vi "Check Action.vi"(6 "HRS Time":dbl, 7 "Values In":dbl[](array[numeric]), 8 "error in (no error)":errorcluster, 11 "Valve in":refnum<class "BangBangControl.lvclass">) -> (0 "error out":errorcluster, 2 "Actions":T1[](array[typedef]), 3 "Valve out":refnum<class "BangBangControl.lvclass">, 5 "Values":dbl[](array[numeric]))   [LabVIEW 2020, in "VolatusControl.lvlib" / "BangBangControl.lvclass"]
uses:
  BangBangControl.lvclass
  Control Action.ctl
  Volatus/MessageQ/MessageQ.lvclass
  BangBangControl.lvclass/BangBangControl.ctl
  State.ctl
  PV Calc/PV Calc.lvclass
  VolatusControl.lvlib
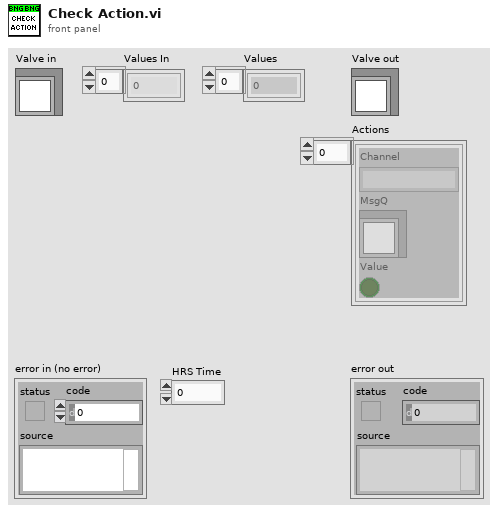
[diagram p1: front panel]
types:
  T1 = typedef "VolatusControl.lvlib/Control Action.ctl" = cluster{"Channel":string, "MsgQ":refnum<class "MessageQ.lvclass">, "Value":bool}
  T2 = typedef "VolatusControl.lvlib/BangBangControl.lvclass/State.ctl" = enum16{"Idle", "RampUp", "RampDown", "Hold", "Disable", "Enable"}
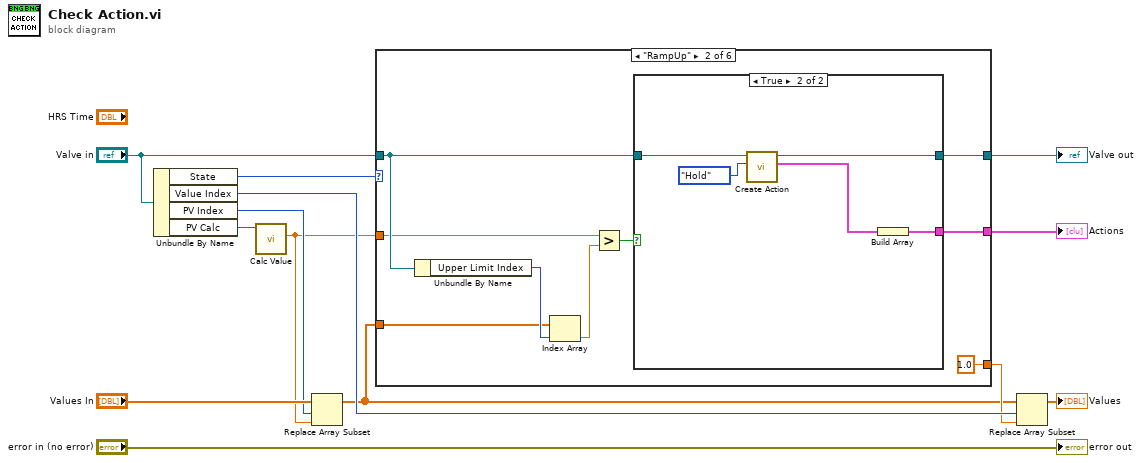
[diagram p0: block diagram]
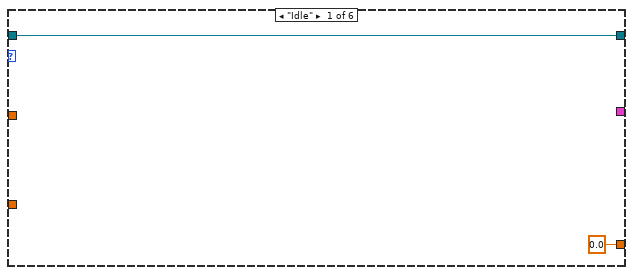
[diagram p2: hidden frame]
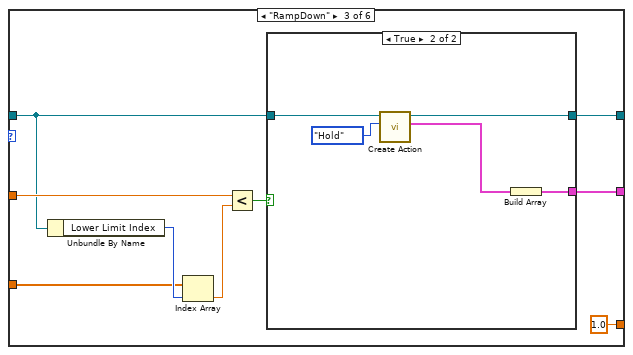
[diagram p4: hidden frame]
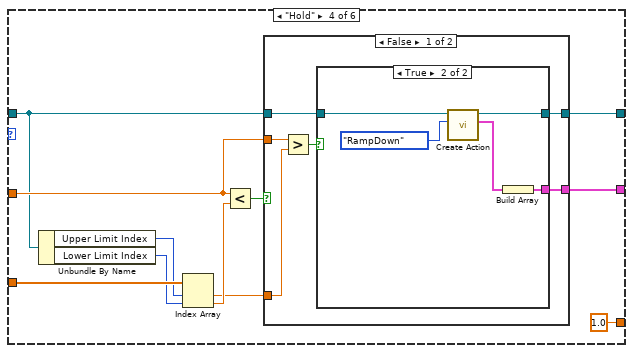
[diagram p6: hidden frame]
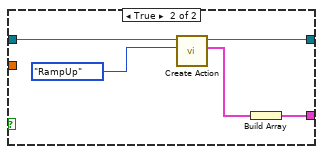
[diagram p8: hidden frame]
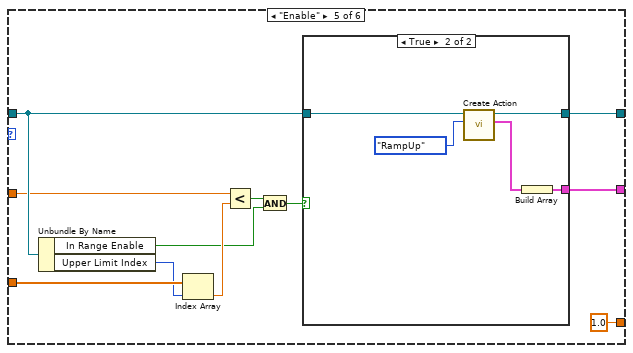
[diagram p9: hidden frame]
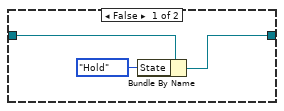
[diagram p10: hidden frame]
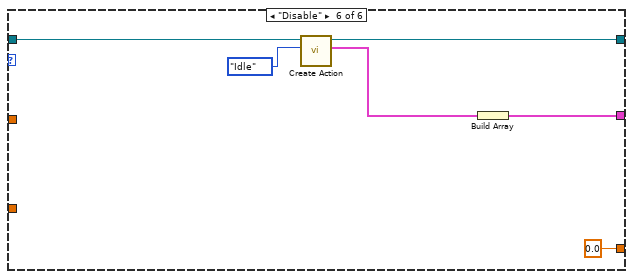
[diagram p11: hidden frame]
diagram:
  n1 = Unbundle By Name("Valve in") -> ("State"=w10:T2, "Value Index"=w11:i32, "PV Index"=w2:i32, "PV Calc"=w4:refnum<class "PV Calc.lvclass">)
  n2 = call "Calc Value.vi"("PV Calc in"=w4) -> ("Value"=w1:dbl)  [unwired: 8 in, 2 out]
  n3 = Replace Array Subset(array="Values In", new element=w1, index=w2) -> (w3:dbl[])
  n4 = case shown="\"RampUp\"" w10 {
    tunnel: w3 -> [_ w22 w38 w55 w82 _]
    tunnel: [0.0 1.0 1.0 1.0 1.0 0.0] -> w8
    tunnel: "Valve in" -> [w14 w24 w31 w46 w83 w97]
    tunnel: [w14 w18 w34 w50 w79 w96] -> w6
    tunnel: [_ w17 w33 w49 w78 w93] -> w5
    tunnel: w1 -> [_ w16 w32 w47 w74 _]
    frame "Idle" {
    }
    frame "RampUp" {
      n5 = Unbundle By Name(w24) -> ("Upper Limit Index"=w23:i32)
      n6 = Index Array(array=w22, index=w23) -> (element=w20:dbl)
      n7 = Greater?(x=w16, y=w20) -> (0:w19:bool)
      n8 = case shown="True" w19 {
        tunnel: w24 -> [w25 w30]
        tunnel: [w25 w29] -> w18
        tunnel: [_ w26] -> w17
        frame False {
        }
        frame True {
          n9 = call "Create Action.vi"("State"=State."Hold", "BangBangControl in"=w30) -> ("Action"=w27:T1, "BangBangControl out"=w29:refnum<class "BangBangControl.lvclass">)  [unwired: 7 in, 1 out]
          n10 = Build Array(w27) -> (w26:T1[])
        }
      }
    }
    frame "RampDown" {
      n11 = Unbundle By Name(w31) -> ("Lower Limit Index"=w39:i32)
      n12 = Index Array(array=w38, index=w39) -> (element=w36:dbl)
      n13 = Less?(x=w32, y=w36) -> (x < y?=w35:bool)
      n14 = case shown="True" w35 {
        tunnel: w31 -> [w40 w45]
        tunnel: [w40 w44] -> w34
        tunnel: [_ w41] -> w33
        frame False {
        }
        frame True {
          n15 = call "Create Action.vi"("State"=State."Hold", "BangBangControl in"=w45) -> ("Action"=w42:T1, "BangBangControl out"=w44:refnum<class "BangBangControl.lvclass">)  [unwired: 7 in, 1 out]
          n16 = Build Array(w42) -> (w41:T1[])
        }
      }
    }
    frame "Hold" {
      n17 = Unbundle By Name(w46) -> ("Upper Limit Index"=w53:i32, "Lower Limit Index"=w54:i32)
      n18 = Index Array(array=w55, index #1=w53, index #2=w54) -> (element #1=w48:dbl, element #2=w52:dbl)
      n19 = Less?(x=w47, y=w52) -> (x < y?=w51:bool)
      n20 = case shown="False" w51 {
        tunnel: w46 -> [w60 w71]
        tunnel: [w58 w73] -> w50
        tunnel: [w57 w69] -> w49
        tunnel: w48 -> [w61 _]
        tunnel: w47 -> [w62 _]
        frame False {
          n21 = Greater?(x=w62, y=w61) -> (0:w59:bool)
          n22 = case shown="True" w59 {
            tunnel: w60 -> [w63 w66]
            tunnel: [w63 w68] -> w58
            tunnel: [_ w64] -> w57
            frame False {
            }
            frame True {
              n23 = call "Create Action.vi"("State"=State."RampDown", "BangBangControl in"=w66) -> ("Action"=w67:T1, "BangBangControl out"=w68:refnum<class "BangBangControl.lvclass">)  [unwired: 7 in, 1 out]
              n24 = Build Array(w67) -> (w64:T1[])
            }
          }
        }
        frame True {
          n25 = call "Create Action.vi"("State"=State."RampUp", "BangBangControl in"=w71) -> ("Action"=w72:T1, "BangBangControl out"=w73:refnum<class "BangBangControl.lvclass">)  [unwired: 7 in, 1 out]
          n26 = Build Array(w72) -> (w69:T1[])
        }
      }
    }
    frame "Enable" {
      n27 = Unbundle By Name(w83) -> ("In Range Enable"=w75:bool, "Upper Limit Index"=w81:i32)
      n28 = Index Array(array=w82, index=w81) -> (element=w77:dbl)
      n29 = Less?(x=w74, y=w77) -> (x < y?=w80:bool)
      n30 = And(x=w80, y=w75) -> (x .and. y?=w76:bool)
      n31 = case shown="True" w76 {
        tunnel: w83 -> [w87 w90]
        tunnel: [w86 w92] -> w79
        tunnel: [_ w88] -> w78
        frame False {
          n32 = Bundle By Name(cluster=w87, "State"=State."Hold") -> (w86:refnum<class "BangBangControl.lvclass">)
        }
        frame True {
          n33 = call "Create Action.vi"("State"=State."RampUp", "BangBangControl in"=w90) -> ("Action"=w91:T1, "BangBangControl out"=w92:refnum<class "BangBangControl.lvclass">)  [unwired: 7 in, 1 out]
          n34 = Build Array(w91) -> (w88:T1[])
        }
      }
    }
    frame "Disable" {
      n35 = call "Create Action.vi"("State"=State."Idle", "BangBangControl in"=w97) -> ("Action"=w94:T1, "BangBangControl out"=w96:refnum<class "BangBangControl.lvclass">)  [unwired: 7 in, 1 out]
      n36 = Build Array(w94) -> (w93:T1[])
    }
  }
  "Valve out" <- w6
  "Actions" <- w5
  n37 = Replace Array Subset(array=w3, new element=w8, index=w11) -> (→"Values":dbl[])
  "error out" <- "error in (no error)"
